vi "Day 25.vi"() -> ()   [LabVIEW 2021]
uses:
  <vilib>/Utility/file.llb/Read Delimited Spreadsheet (string).vi
panel:
  out "Character Array":string[][](array[string])
  out "x+1":i32
  in  "Input File":enum32{"example input", "input"}(radio)
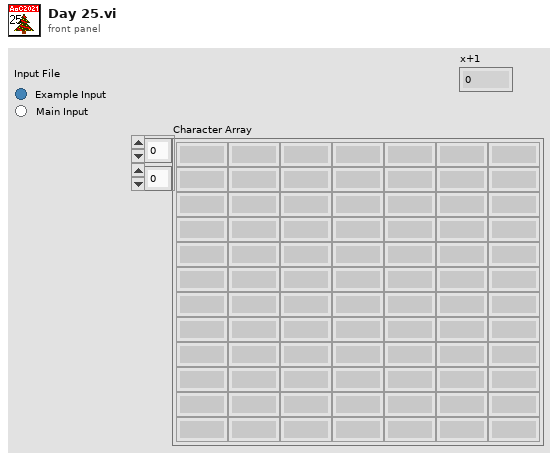
[diagram p1: front panel]
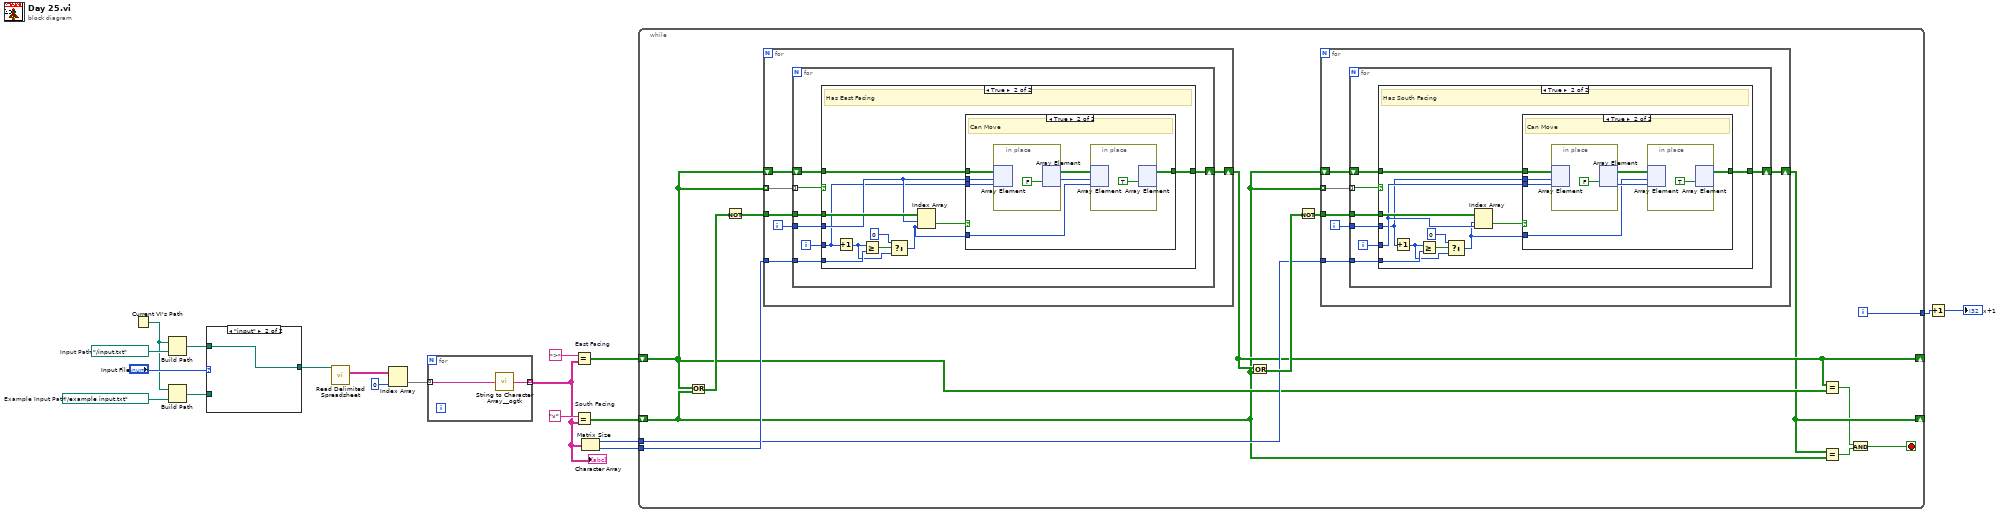
[diagram p0: block diagram]
diagram:
  w18 = path "../example input.txt"  # Example Input Path
  w19 = path "../input.txt"  # Input Path
  n1 = Current VI's Path() -> (path=w13:path)
  n2 = Build Path(base path=w13, name or relative path=w19) -> (appended path=w16:path)
  n3 = Build Path(base path=w13, name or relative path=w18) -> (appended path=w15:path)
  n4 = case shown="\"input\"" "Input File" {
    tunnel: w16 -> [_ w21]
    tunnel: w15 -> [w20 _]
    tunnel: [w20 w21] -> w14
    frame "example input" {
    }
    frame "input" {
    }
  }
  n5 = call-poly <vilib>:"Read Delimited Spreadsheet.vi"("file path (dialog if empty)"=w14) -> ("all rows"=w12:string[][])  [unwired: 9 in, 5 out]
  n6 = Index Array(array=w12, index (col)=0 ("disabled index (col)")) -> (element=w10:string[])  [unwired: 1 in]
  n7 = for {
    tunnel: w10 -> [w23] mode=indexing
    tunnel: [w22] -> w5 mode=indexing
    n8 = call <userlib>:"String to Character Array__ogtk.vi"("Input String"=w23) -> ("Character Array"=w22:string[])
  }
  "Character Array" <- w5
  n9 = Equal? "East Facing"(x=">", y=w5) -> (x = y?=w7:bool[][])
  n10 = Equal? "South Facing"(x="v", y=w5) -> (x = y?=w6:bool[][])
  n11 = Matrix Size(0:w5) -> (1:w4:i32, 2:w3:i32)
  n12 = while {
    shift-right: [w33] -> _
    shift-left: w7 -> [w32]
    shift-right: [w31] -> _
    shift-left: w6 -> [w30]
    tunnel: w4 -> [w34]
    tunnel: w3 -> [w36]
    tunnel: [w26] -> w2
    i -> [w26]
    stop <- w27 stop-if-true
    n13 = Or(x=w32, y=w30) -> (x .or. y?=w37:bool[][])
    n14 = Not(x=w37) -> (.not. x?=w25:bool[][])
    n15 = for {
      tunnel: w32 -> [w78] mode=indexing
      tunnel: w25 -> [w77]
      tunnel: w36 -> [w75]
      shift-right: [w73] -> w33
      shift-left: w32 -> [w74]
      i -> [w76]
      n16 = for {
        tunnel: w78 -> [w80] mode=indexing
        tunnel: w77 -> [w84]
        tunnel: w76 -> [w81]
        tunnel: w75 -> [w85]
        shift-right: [w79] -> w73
        shift-left: w74 -> [w82]
        i -> [w83]
        n17 = case shown="True" w80 {
          tunnel: w85 -> [_ w97]
          tunnel: w84 -> [_ w93]
          tunnel: w83 -> [_ w89]
          tunnel: w82 -> [w86 w92]
          tunnel: w81 -> [_ w91]
          tunnel: [w86 w87] -> w79
          frame False {
          }
          frame True {
            # "Has East Facing"
            n18 = Increment(x=w89) -> (x+1=w95:i32)
            n19 = Greater Or Equal?(x=w95, y=w97) -> (x >= y?=w96:bool)
            n20 = Select(t=0, s=w96, f=w95) -> (s? t:f=w88:i32)
            n21 = Index Array(array=w93, index (row)=w91, index (col)=w88) -> (element=w90:bool)
            n22 = case shown="True" w90 {
              tunnel: w92 -> [w98 w105]
              tunnel: w91 -> [_ w104]
              tunnel: w89 -> [_ w102]
              tunnel: w88 -> [_ w100]
              tunnel: [w98 w99] -> w87
              frame False {
              }
              frame True {
                # "Can Move"
                n23 = in-place {
                  n24 = in-place-array #1(w105, w104, w102) -> ()  [unwired: 1 out]
                  n25 = in-place-array #1(FALSE) -> (w103:bool[][], w101:i32)  [unwired: 1 out]
                }
                n26 = in-place {
                  n27 = in-place-array #2(w103, w101, w100) -> ()  [unwired: 1 out]
                  n28 = in-place-array #2(TRUE) -> (w99:bool[][])  [unwired: 2 out]
                }
              }
            }
          }
        }
      }
    }
    n29 = Or(x=w33, y=w30) -> (x .or. y?=w35:bool[][])
    n30 = Not(x=w35) -> (.not. x?=w24:bool[][])
    n31 = for {
      tunnel: w30 -> [w43] mode=indexing
      tunnel: w24 -> [w42]
      tunnel: w34 -> [w40]
      shift-right: [w38] -> w31
      shift-left: w30 -> [w39]
      i -> [w41]
      n32 = for {
        tunnel: w43 -> [w45] mode=indexing
        tunnel: w42 -> [w49]
        tunnel: w41 -> [w46]
        tunnel: w40 -> [w50]
        shift-right: [w44] -> w38
        shift-left: w39 -> [w47]
        i -> [w48]
        n33 = case shown="True" w45 {
          tunnel: w50 -> [_ w62]
          tunnel: w49 -> [_ w58]
          tunnel: w48 -> [_ w54]
          tunnel: w47 -> [w51 w57]
          tunnel: w46 -> [_ w53]
          tunnel: [w51 w55] -> w44
          frame False {
          }
          frame True {
            # "Has South Facing"
            n34 = Increment(x=w53) -> (x+1=w60:i32)
            n35 = Greater Or Equal?(x=w60, y=w62) -> (x >= y?=w61:bool)
            n36 = Select(t=0, s=w61, f=w60) -> (s? t:f=w52:i32)
            n37 = Index Array(array=w58, index (row)=w52, index (col)=w54) -> (element=w56:bool)
            n38 = case shown="True" w56 {
              tunnel: w57 -> [w63 w70]
              tunnel: w53 -> [_ w69]
              tunnel: w54 -> [_ w67]
              tunnel: w52 -> [_ w64]
              tunnel: [w63 w66] -> w55
              frame False {
              }
              frame True {
                # "Can Move"
                n39 = in-place {
                  n40 = in-place-array #3(w70, w69, w67) -> ()  [unwired: 1 out]
                  n41 = in-place-array #3(FALSE) -> (w68:bool[][], w65:i32)  [unwired: 1 out]
                }
                n42 = in-place {
                  n43 = in-place-array #4(w68, w64, w65) -> ()  [unwired: 1 out]
                  n44 = in-place-array #4(TRUE) -> (w66:bool[][])  [unwired: 2 out]
                }
              }
            }
          }
        }
      }
    }
    n45 = Equal?(x=w33, y=w32) -> (x = y?=w29:bool)
    n46 = Equal?(x=w31, y=w30) -> (x = y?=w28:bool)
    n47 = And(x=w29, y=w28) -> (x .and. y?=w27:bool)
  }
  n48 = Increment(x=w2) -> (x+1=→"x+1":i32)
